vi "Create InstrumentStudio Plug-In.vi"() -> ()   [LabVIEW 2021, in "InstrumentStudio Plug-In Editor.lvlib"]
doc: "Tool to generate InstrumentStudio plug-in from template."
uses:
  _InstrumentStudio Plug-In Editor/InstrumentStudio Plug-In Editor.lvlib
  <vilib>/Utility/error.llb/ErrWarn.ctl
  _InstrumentStudio Plug-In Editor/Plugin Configuration.ctl
panel:
  in  "Group":string caption="InstrumentStudio Plug-in Group"
  out "Status":T1=TRUE caption="InstrumentStudio plug-in name must be unique and cannot contain any of the following characters:\n           \\ / : * ? \" < > |"
  in  "Create InstrumentStudio Plug-in":bool
  in  "Name":string caption="InstrumentStudio Plug-in Name"
  out "Active Project Name":string
  # "* Project in which the InstrumentStudio plug-in will be created"
  # "* Group under which the plug-in will be populated in the Add-Ons\ncategory of InstrumentStudio's Edit Layout Dialog"
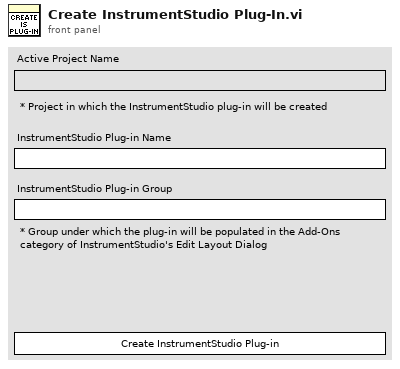
[diagram p1: front panel]
types:
  T1 = typedef "ErrWarn.ctl" = bool
  T2 = enum8{"Enabled", "Disabled", "Disabled and Grayed Out"}
  T3 = typedef "InstrumentStudio Plug-In Editor.lvlib/Plugin Configuration.ctl" = cluster{"project refnum":refnum<vi>, "plugin name":string, "plugin group name":string}
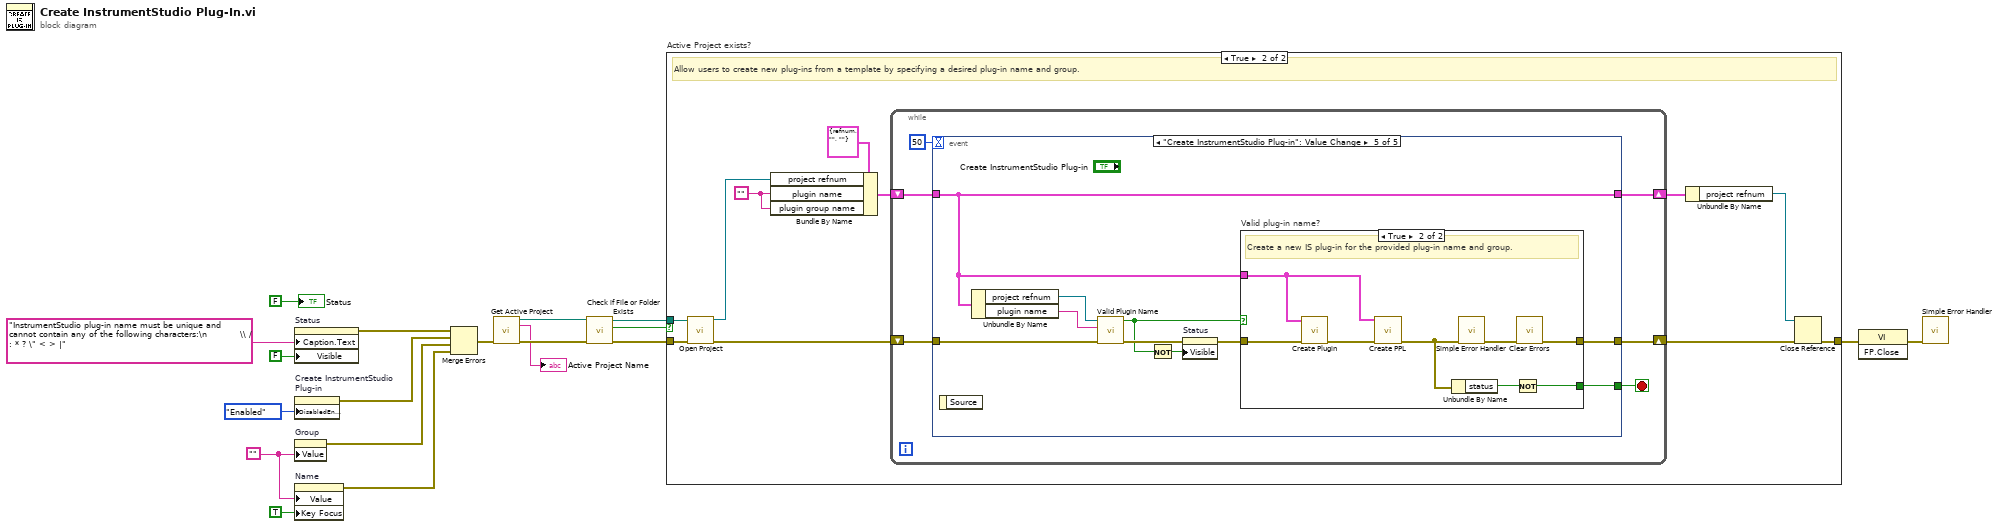
[diagram p0: block diagram]
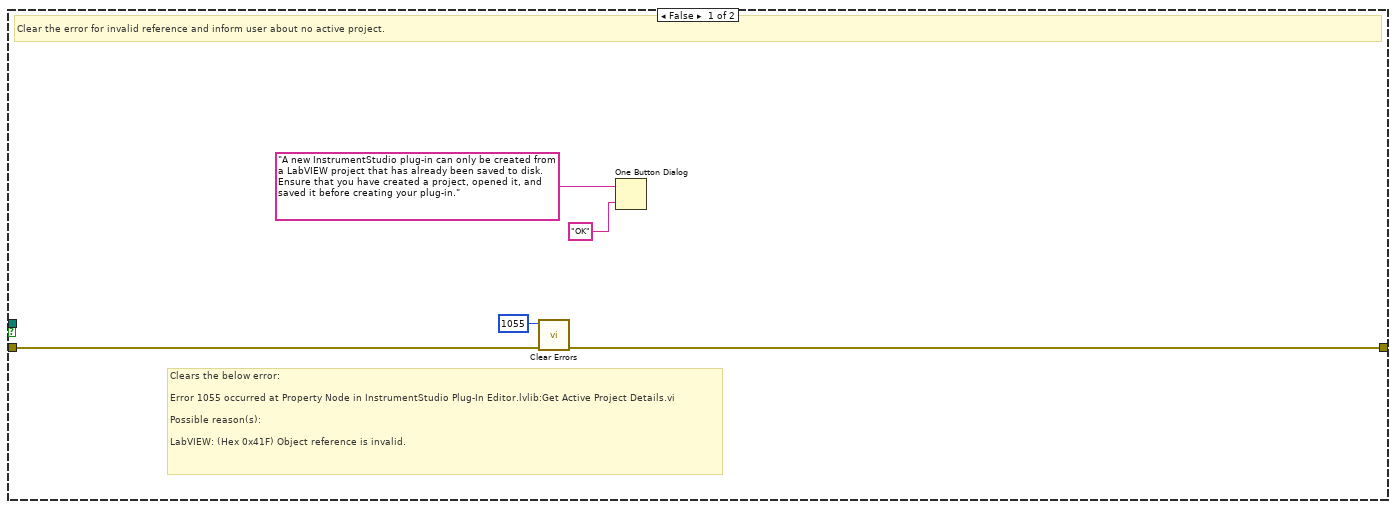
[diagram p2: hidden frame]
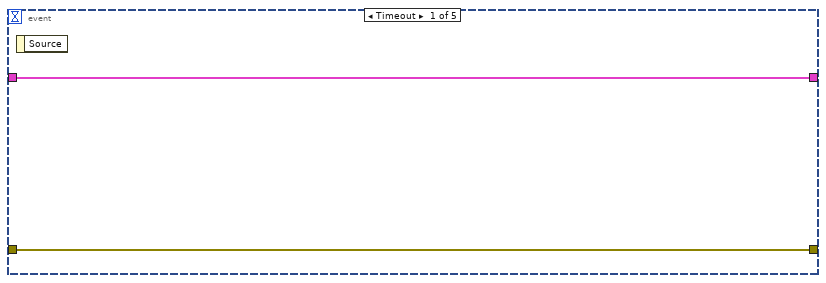
[diagram p3: hidden frame]
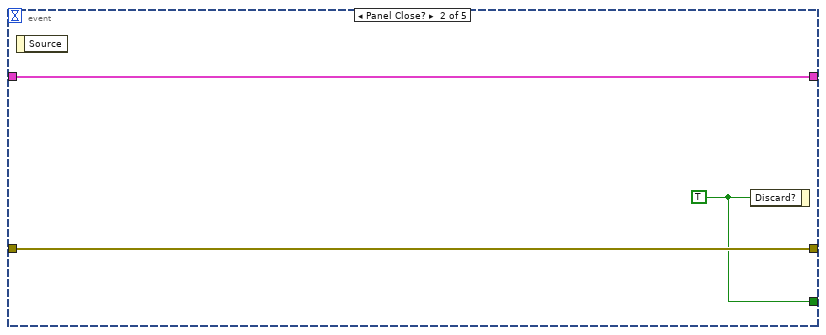
[diagram p4: hidden frame]
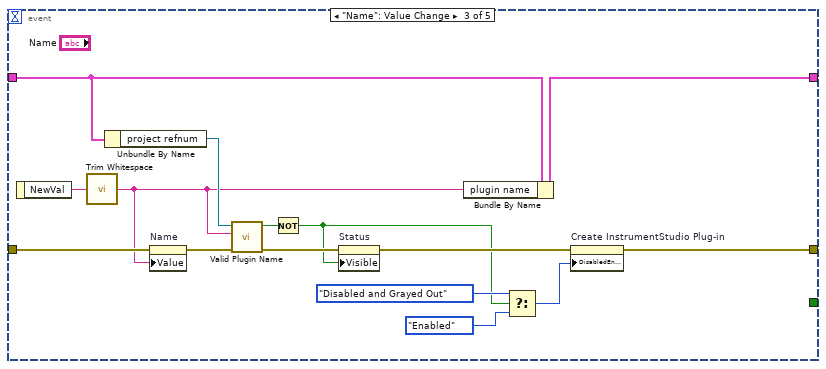
[diagram p5: hidden frame]
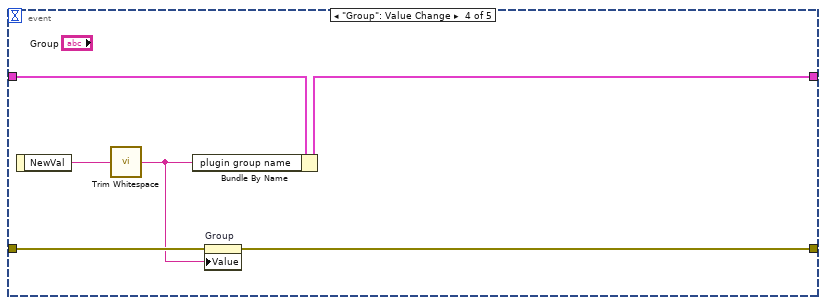
[diagram p6: hidden frame]
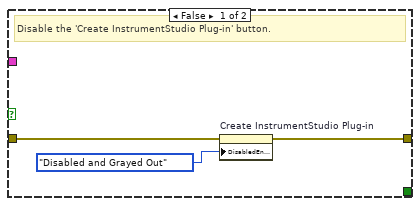
[diagram p7: hidden frame]
diagram:
  w2 = "" ("Group")
  n1 = property on="Status" class="Bool"("Caption.Text"="InstrumentStudio plug-in name must be unique and cannot contain any of the following characters:\n           \\ / : * ? \" < > |" ("Status"), "Visible"=FALSE) -> (error out=w12:errorcluster)  [unwired: 2 in, 1 out]
  n2 = property on="Create InstrumentStudio\nPlug-in" class="Bool"("DisabledEnum"=T2."Enabled" ("Disabled")) -> (error out=w11:errorcluster)  [unwired: 2 in, 1 out]
  n3 = property on="Group" class="Str"("Value"=w2) -> (error out=w10:errorcluster)  [unwired: 2 in, 1 out]
  n4 = property on="Name" class="Str"("Value"=w2, "Key Focus"=TRUE) -> (error out=w9:errorcluster)  [unwired: 2 in, 1 out]
  n5 = Merge Errors(w12, w11, w10, w9) -> (w8:errorcluster)
  n6 = call "Get Active Project.vi"("error in"=w8) -> ("path"=w14:path, "name"=→"Active Project Name":string, "error out"=w15:errorcluster)  [unwired: 12 in]
  n7 = call <vilib>:"Check if File or Folder Exists.vi"("error in (no error)"=w15, "path"=w14) -> ("error out"=w17:errorcluster, "file or folder exists?"=w1:bool, "dup path"=w16:path)  [unwired: 7 in]
  n8 = case "Active Project exists?" shown="True" w1 {
    tunnel: w17 -> [w23 w34]
    tunnel: [w22 w27] -> w18
    tunnel: w16 -> [_ w26]
    frame False {
      # "Clears the below error:\n\nError 1055 occurred at Property Node in InstrumentStudio Plug-In Editor.lvlib:Get Active Project Details.vi\n\nPossible reason(s):\n\nLabVIEW: (Hex 0x41F) Object reference is invalid."
      # "Clear the error for invalid reference and inform user about no active project."
      n9 = call <vilib>:"Clear Errors.vi"("error in (no error)"=w23, "specific error code to clear (0: all)"=1055) -> ("error out"=w22:errorcluster)  [unwired: 4 in, 1 out]
      n10 = One Button Dialog(message="A new InstrumentStudio plug-in can only be created from a LabVIEW project that has already been saved to disk.  Ensure that you have created a project, opened it, and saved it before creating your plug-in.", button name ("OK")="OK") -> ()  [unwired: 1 out]
    }
    frame True {
      w25 = ""
      # "Allow users to create new plug-ins from a template by specifying a desired plug-in name and group."
      n11 = call "Open Project.vi"("project path"=w26, "error in"=w34) -> ("project refnum"=w32:refnum<vi>, "error out"=w35:errorcluster)  [unwired: 12 in]
      n12 = Bundle By Name(cluster=T3 {"project refnum"=refnum, "plugin name"="", "plugin group name"=""}, "project refnum"=w32, "plugin name"=w25, "plugin group name"=w25) -> (w31:T3)
      n13 = while {
        shift-right: [w38] -> w28
        shift-left: w35 -> [w41]
        shift-right: [w39] -> w30
        shift-left: w31 -> [w40]
        stop <- w36 stop-if-true
        n14 = event shown="[4] \"Create InstrumentStudio Plug-in\": Value Change" {
          selector: _ -> [_ _ _ _ _]
          dyn-events: _ -> [_ _ _ _ _]
          timeout: 50 -> [_ _ _ _ _]
          tunnel: w41 -> [w42 w45 w55 w65 w77]
          tunnel: w40 -> [w43 w46 w59 w67 w72]
          tunnel: [w43 w46 w60 w66 w72] -> w39
          tunnel: [w42 w45 w52 w64 w74] -> w38
          tunnel: [_ w44 _ _ w68] -> w36
          event Timeout {
            n15 = event-data() -> ()  [unwired: 1 in, 1 out]
          }
          event Panel Close? {
            w44 = TRUE ("Discard?")
            n16 = event-data() -> ()  [unwired: 1 in, 1 out]
            n17 = event-data("Discard?"=w44) -> ()  [unwired: 1 in, 1 out]
          }
          event "Name": Value Change {
            n18 = event-data() -> ("NewVal"=w61:string)  [unwired: 1 in]
            n19 = call <vilib>:"Trim Whitespace.vi"("string"=w61) -> ("trimmed string"=w54:string)  [unwired: 1 in]
            n20 = Unbundle By Name(w59) -> ("project refnum"=w58:refnum<vi>)
            n21 = property on="Name" class="Str"(error in=w55, "Value"=w54) -> (error out=w56:errorcluster)  [unwired: 1 in, 1 out]
            n22 = call "Valid Plugin Name.vi"("error in"=w56, "requested plugin name"=w54, "project refnum"=w58) -> ("error out"=w57:errorcluster, "valid name?"=w53:bool)  [unwired: 7 in]
            n23 = Not(x=w53) -> (.not. x?=w47:bool)
            n24 = property on="Status" class="Bool"(error in=w57, "Visible"=w47) -> (error out=w51:errorcluster)  [unwired: 1 in, 1 out]
            n25 = Bundle By Name(cluster=w59, "plugin name"=w54) -> (w60:T3)
            n26 = Select(t=T2."Disabled and Grayed Out" ("Disabled"), s=w47, f=T2."Enabled" ("Disabled")) -> (s? t:f=w48:T2)
            n27 = property on="Create InstrumentStudio Plug-in" class="Bool"(error in=w51, "DisabledEnum"=w48) -> (error out=w52:errorcluster)  [unwired: 1 in, 1 out]
          }
          event "Group": Value Change {
            n28 = event-data() -> ("NewVal"=w63:string)  [unwired: 1 in]
            n29 = call <vilib>:"Trim Whitespace.vi"("string"=w63) -> ("trimmed string"=w62:string)  [unwired: 1 in]
            n30 = Bundle By Name(cluster=w67, "plugin group name"=w62) -> (w66:T3)
            n31 = property on="Group" class="Str"(error in=w65, "Value"=w62) -> (error out=w64:errorcluster)  [unwired: 1 in, 1 out]
          }
          event "Create InstrumentStudio Plug-in": Value Change {
            n32 = event-data() -> ()  [unwired: 1 in, 1 out]
            n33 = Unbundle By Name(w72) -> ("project refnum"=w70:refnum<vi>, "plugin name"=w73:string)
            n34 = call "Valid Plugin Name.vi"("error in"=w77, "requested plugin name"=w73, "project refnum"=w70) -> ("error out"=w76:errorcluster, "valid name?"=w69:bool)  [unwired: 7 in]
            n35 = Not(x=w69) -> (.not. x?=w71:bool)
            n36 = property on="Status" class="Bool"(error in=w76, "Visible"=w71) -> (error out=w75:errorcluster)  [unwired: 1 in, 1 out]
            n37 = case "Valid plug-in name?" shown="True" w69 {
              tunnel: w75 -> [w80 w88]
              tunnel: [w79 w84] -> w74
              tunnel: w72 -> [_ w82]
              tunnel: [_ w81] -> w68
              frame False {
                # "Disable the 'Create InstrumentStudio Plug-in' button."
                n38 = property on="Create InstrumentStudio Plug-in" class="Bool"(error in=w80, "DisabledEnum"=T2."Disabled and Grayed Out" ("Disabled")) -> (error out=w79:errorcluster)  [unwired: 1 in, 1 out]
              }
              frame True {
                # "Create a new IS plug-in for the provided plug-in name and group."
                n39 = call "Create Plugin.vi"("error in"=w88, "configuration"=w82) -> ("error out"=w87:errorcluster)  [unwired: 9 in]
                n40 = call "Create PPL.vi"("configuration"=w82, "error in"=w87) -> ("error out"=w86:errorcluster)  [unwired: 13 in]
                n41 = Unbundle By Name(w86) -> ("status"=w83:bool)
                n42 = call <vilib>:"Simple Error Handler.vi"("error in (no error)"=w86) -> ("error out"=w85:errorcluster)  [unwired: 4 in, 4 out]
                n43 = Not(x=w83) -> (.not. x?=w81:bool)
                n44 = call <vilib>:"Clear Errors.vi"("error in (no error)"=w85) -> ("error out"=w84:errorcluster)  [unwired: 5 in, 1 out]
              }
            }
          }
        }
      }
      n45 = Unbundle By Name(w30) -> ("project refnum"=w29:refnum<vi>)
      n46 = Close Reference(reference=w29, error in (no error)=w28) -> (error out=w27:errorcluster)
    }
  }
  n47 = invoke class="VI" method="FP.Close"(error in=w18) -> (error out=w19:errorcluster)  [unwired: 2 in, 2 out]
  n48 = call <vilib>:"Simple Error Handler.vi"("error in (no error)"=w19) -> ()  [unwired: 4 in, 5 out]
  "Status" <- T1 FALSE ("Status")
